vi "Ramsey_Tau_manipulation.vi"(8 "Dont Invert?":bool, 9 "Numeric 2":i32, 10 "Numeric":i32, 11 "Step Size":dbl format="%#_13g") -> (2 "x+y":dbl)   [LabVIEW 2024]
uses:
  <vilib>/Utility/error.llb/DialogTypeEnum.ctl
  SpinCore_API_file_location.vi
panel:
  out "x+y 4":dbl
  out "x+y 3":dbl
  out "output array 2":T1(array[cluster])
  out "output array":T1(array[cluster])
  in  "Instructions":T1(array[cluster])=[{"Instruct Data"=0, "Op Code"=0, "Flags"=[FALSE, FALSE, TRUE, FALSE, FALSE, FALSE, FALSE, TRUE, FALSE, FALSE, FALSE, FALSE, FALSE, FALSE, FALSE, FALSE, FALSE, FALSE, FALSE, FALSE, FALSE, FALSE, FALSE, TRUE], "Comments"="0 triggers", "Time (s)"=1e-07}, {"Instruct Data"=0, "Op Code"=0, "Flags"=[FALSE, FALSE, FALSE, FALSE, FALSE, FALSE, FALSE, TRUE, FALSE, FALSE, FALSE, FALSE, FALSE, FALSE, FALSE, FALSE, FALSE, FALSE, FALSE, FALSE, FALSE, FALSE, FALSE, FALSE], "Comments"="1Dark", "Time (s)"=6e-06}, {"Instruct Data"=0, "Op Code"=0, "Flags"=[TRUE, FALSE, FALSE, TRUE, FALSE, FALSE, FALSE, TRUE, FALSE, FALSE, FALSE, FALSE, FALSE, FALSE, FALSE, FALSE, FALSE, FALSE, FALSE, FALSE, FALSE, FALSE, FALSE, FALSE], "Comments"="2 pi/2", "Time (s)"=6.9e-08}, {"Instruct Data"=0, "Op Code"=0, "Flags"=[FALSE, FALSE, FALSE, FALSE, FALSE, FALSE, FALSE, TRUE, FALSE, FALSE, FALSE, FALSE, FALSE, FALSE, FALSE, FALSE, FALSE, FALSE, FALSE, FALSE, FALSE, FALSE, FALSE, FALSE], "Comments"="3 tau", "Time (s)"=1e-08}, {"Instruct Data"=0, "Op Code"=0, "Flags"=[TRUE, FALSE, FALSE, TRUE, FALSE, FALSE, FALSE, TRUE, FALSE, FALSE, FALSE, FALSE, FALSE, FALSE, FALSE, FALSE, FALSE, FALSE, FALSE, FALSE, FALSE, FALSE, FALSE, FALSE], "Comments"="4 pi/2", "Time (s)"=6.9e-08}, {"Instruct Data"=0, "Op Code"=0, "Flags"=[FALSE, TRUE, FALSE, FALSE, FALSE, FALSE, FALSE, TRUE, FALSE, FALSE, FALSE, FALSE, FALSE, FALSE, FALSE, FALSE, FALSE, FALSE, FALSE, FALSE, FALSE, FALSE, FALSE, FALSE], "Comments"="5 AOM Buffer", "Time (s)"=5e-07}, {"Instruct Data"=0, "Op Code"=0, "Flags"=[FALSE, TRUE, FALSE, FALSE, FALSE, FALSE, FALSE, FALSE, FALSE, FALSE, FALSE, FALSE, FALSE, FALSE, FALSE, FALSE, FALSE, FALSE, FALSE, FALSE, FALSE, FALSE, FALSE, FALSE], "Comments"="6 inhibit off", "Time (s)"=5e-07}, {"Instruct Data"=0, "Op Code"=0, "Flags"=[FALSE, TRUE, FALSE, FALSE, FALSE, FALSE, FALSE, TRUE, FALSE, FALSE, FALSE, FALSE, FALSE, FALSE, FALSE, FALSE, FALSE, FALSE, FALSE, FALSE, FALSE, FALSE, FALSE, FALSE], "Comments"="7  AOM", "Time (s)"=6e-06}, {"Instruct Data"=0, "Op Code"=0, "Flags"=[FALSE, FALSE, FALSE, FALSE, FALSE, FALSE, FALSE, TRUE, FALSE, FALSE, FALSE, FALSE, FALSE, FALSE, FALSE, FALSE, FALSE, FALSE, FALSE, FALSE, FALSE, FALSE, FALSE, FALSE], "Comments"="8 Dark", "Time (s)"=5e-06}, {"Instruct Data"=0, "Op Code"=0, "Flags"=[FALSE, TRUE, FALSE, FALSE, FALSE, FALSE, FALSE, TRUE, FALSE, FALSE, FALSE, FALSE, FALSE, FALSE, FALSE, FALSE, FALSE, FALSE, FALSE, FALSE, FALSE, FALSE, FALSE, FALSE], "Comments"="9AOM delay", "Time (s)"=5e-07}, {"Instruct Data"=0, "Op Code"=0, "Flags"=[FALSE, TRUE, FALSE, FALSE, FALSE, FALSE, FALSE, FALSE, FALSE, FALSE, FALSE, FALSE, FALSE, FALSE, FALSE, FALSE, FALSE, FALSE, FALSE, FALSE, FALSE, FALSE, FALSE, FALSE], "Comments"="10 inhibit off", "Time (s)"=5e-07}, {"Instruct Data"=0, "Op Code"=6, "Flags"=[FALSE, TRUE, FALSE, FALSE, FALSE, FALSE, FALSE, TRUE, FALSE, FALSE, FALSE, FALSE, FALSE, FALSE, FALSE, FALSE, FALSE, FALSE, FALSE, FALSE, FALSE, FALSE, FALSE, FALSE], "Comments"="11 AOM", "Time (s)"=6e-06}, {"Instruct Data"=0, "Op Code"=6, "Flags"=[FALSE, FALSE, FALSE, FALSE, FALSE, FALSE, FALSE, FALSE, FALSE, FALSE, FALSE, FALSE, FALSE, FALSE, FALSE, FALSE, FALSE, FALSE, FALSE, FALSE, FALSE, FALSE, FALSE, FALSE], "Comments"="12", "Time (s)"=1e-06}] {"Time (s)" format="%.3p"; "Op Code" items=["Continue", "Stop", "Loop", "End Loop", "JSR", "RTS", "Branch", "Long Delay", "Wait"]}
  in  "# of Instructions":u32=12
  in  "clock_freq (MHz)":dbl=500.0
  # "1)MW\n2)AOM\n3)SR400 Trig\n4) I\n5)Q\n8) Inhibit\n24) Oscillocope trig"
  # "1"
  # "2"
  # "3"
  # "4"
  # "5"
  # "6"
  # "7"
  # "8"
  # "9"
  # "10"
  # "11"
  # "12"
  # "13"
  # "14"
  # "15"
  # "16"
  # "17"
  # "18"
  # "19"
  # "20"
  # "21"
  # "22"
  # "23"
  # "24"
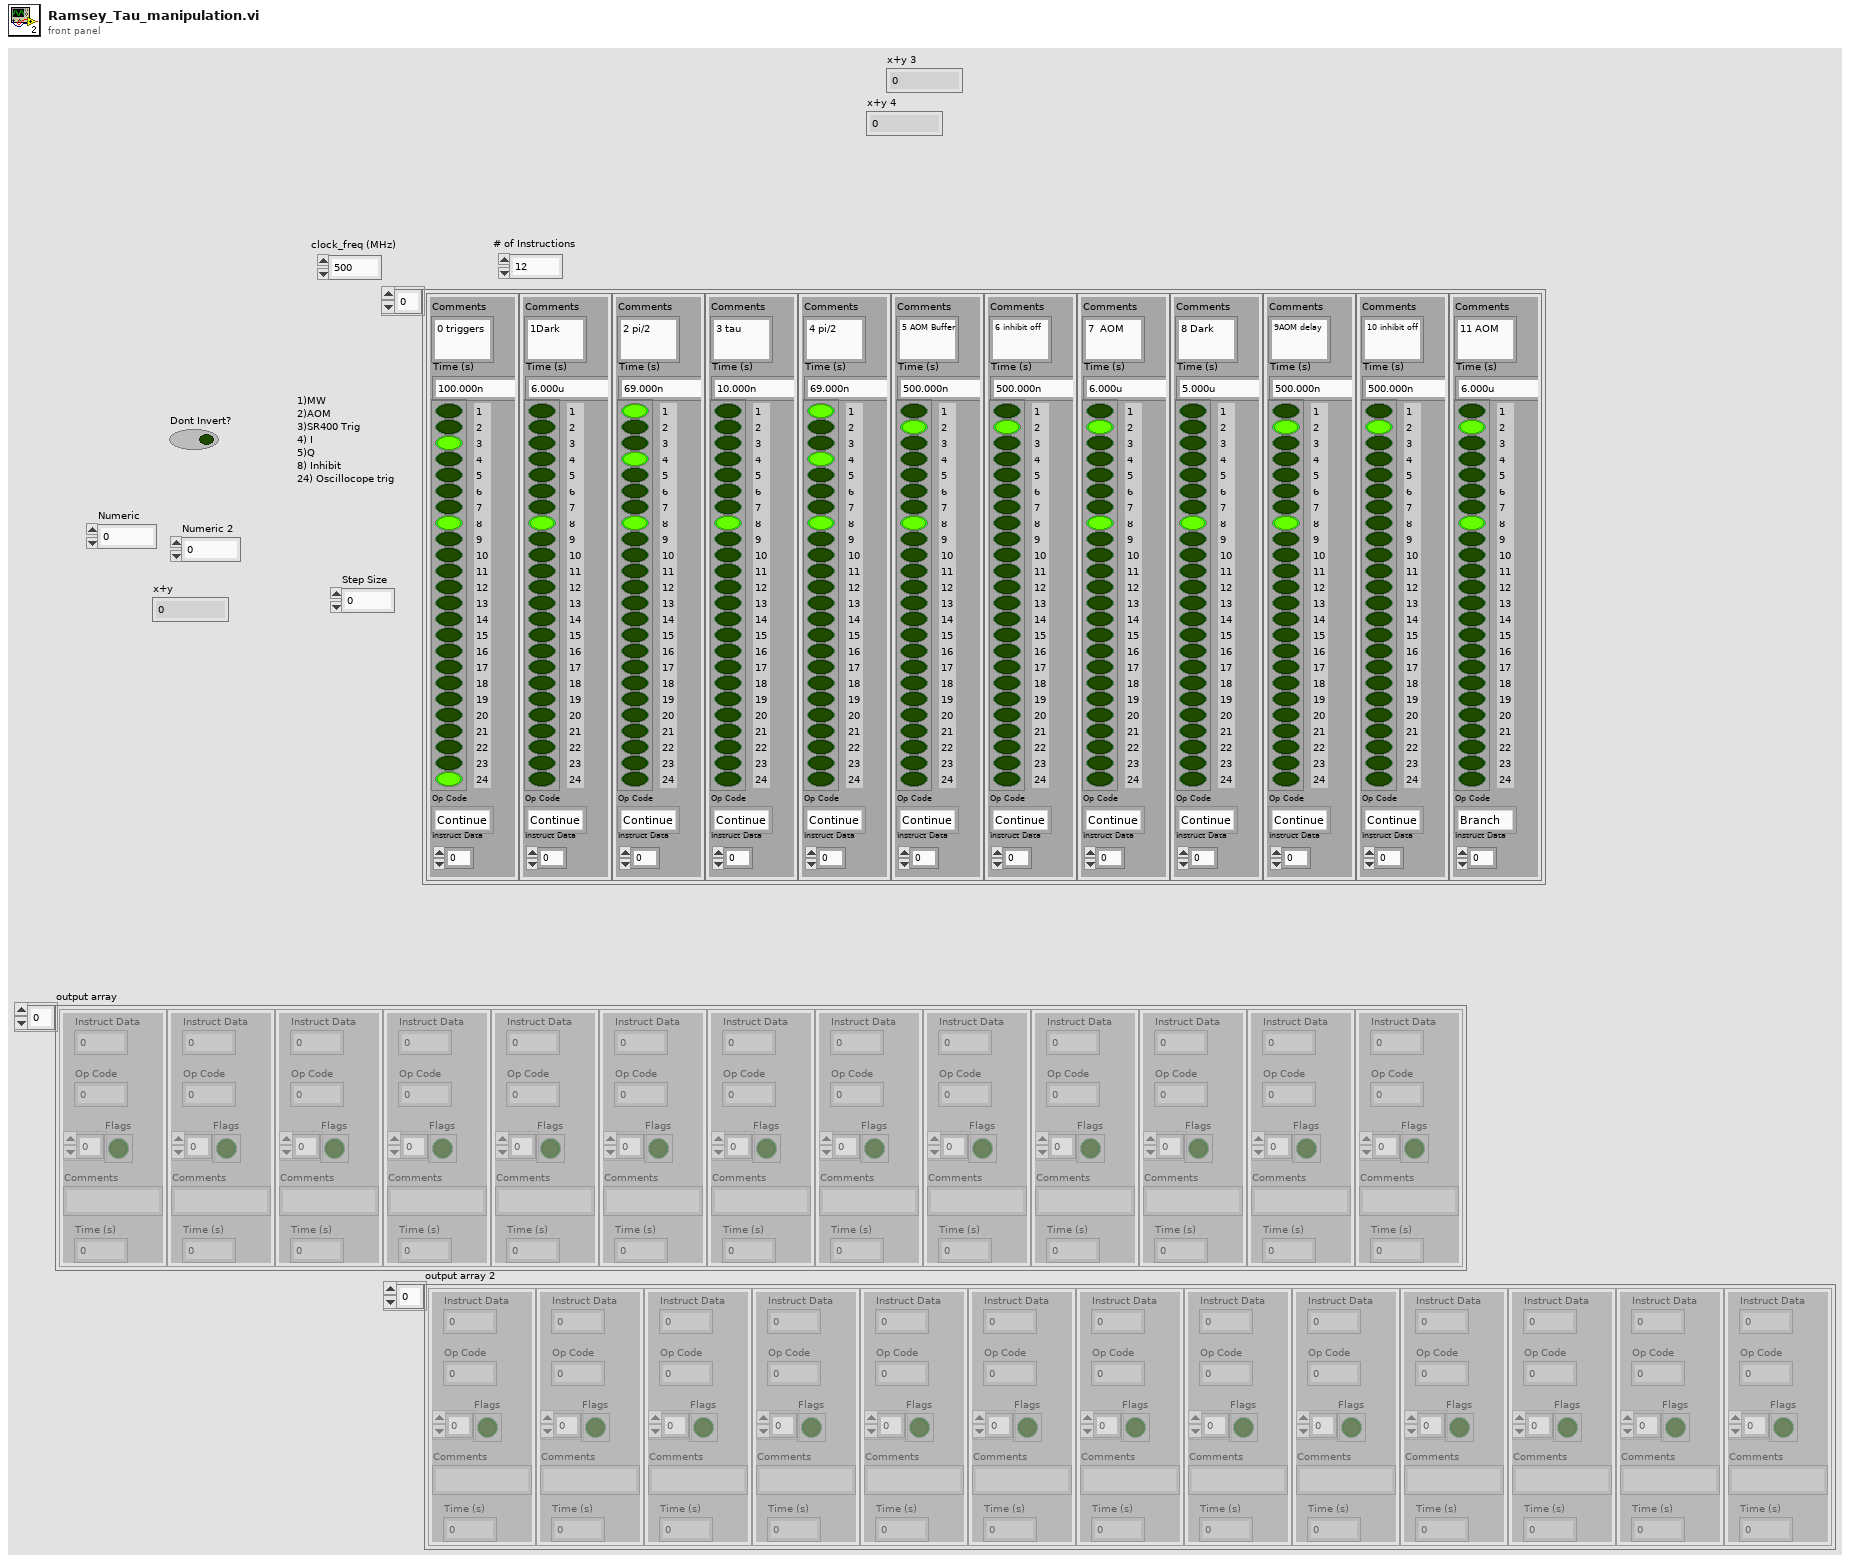
[diagram p1: front panel]
types:
  T1 = cluster{"Instruct Data":i32, "Op Code":i32, "Flags":bool[], "Comments":string, "Time (s)":dbl}[]
  T2 = typedef "DialogTypeEnum.ctl" = enum16{"no dialog", "OK message", "continue or stop message", "auto error handling dialog", "OK message + warnings", "continue/stop + warnings"}
  T3 = enum16{"Pulse Program", "Frequency Registers", "TX Phase Registers", "RX Phase Registers"}
  T4 = cluster{"Instruct Data":i32, "Op Code":i32, "Flags":bool[], "Comments":string, "Time (s)":dbl}
  T5 = cluster{"Instruct Data":i32, "Op Code":i32, "Flags":bool[], "Comments":string, dbl}
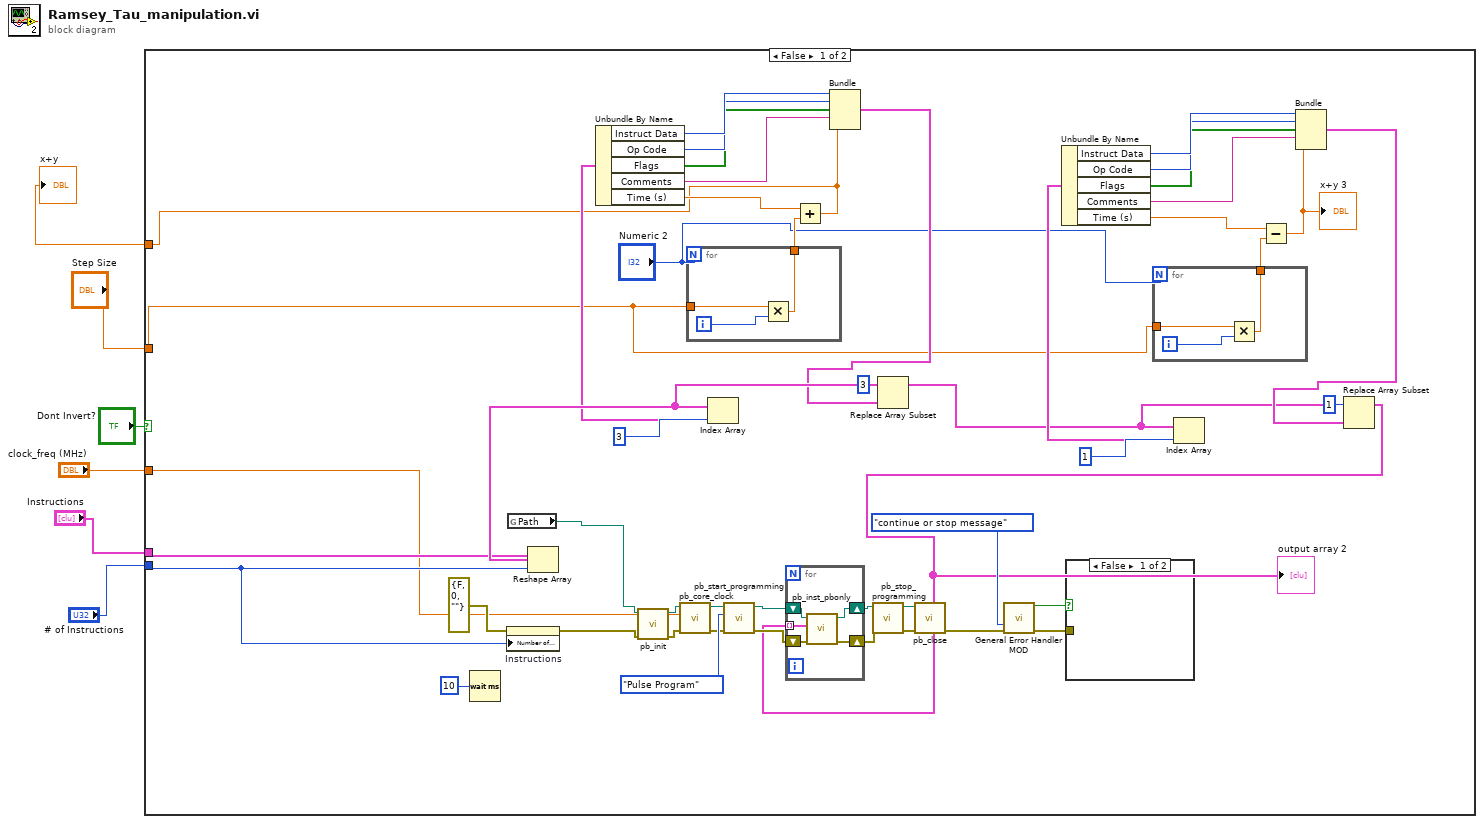
[diagram p0: block diagram]
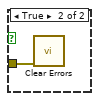
[diagram p2: hidden frame]
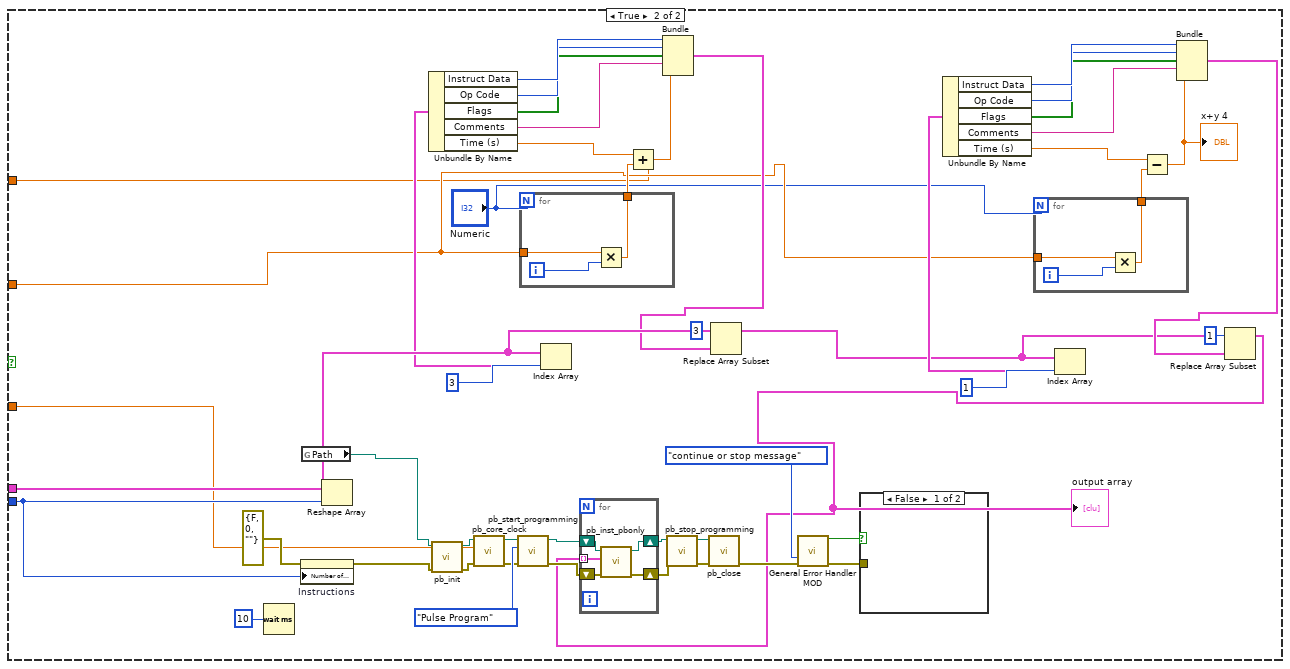
[diagram p3: hidden frame]
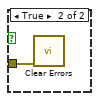
[diagram p4: hidden frame]
diagram:
  n1 = case shown="False" "Dont Invert?" {
    tunnel: "Instructions" -> [w25 w86]
    tunnel: "# of Instructions" -> [w24 w85]
    tunnel: "clock_freq (MHz)" -> [w23 w84]
    tunnel: "Step Size" -> [w9 w72]
    tunnel: [w7 w68] -> w1
    frame False {
      n2 = Wait (ms)(milliseconds to wait=u32 10) -> ()  [unwired: 1 out]
      n3 = property on="Instructions" class="Arr (strict)"(error in=errorcluster {"status"=FALSE, "code"=0, "source"=""} ("error in (no error)"), "Number of Columns"=w24) -> (error out=w30:errorcluster)  [unwired: 1 in, 1 out]
      n4 = global read "SpinCore_API_file_location.vi" "Path"() -> (w31:path)
      n5 = Reshape Array "Reshape Array"(w25, w24) -> (w36:T1)
      n6 = call "pb_init.vi"("error in (no error)"=w30, "path in"=w31) -> ("error out"=w29:errorcluster, "path out"=w28:path)  [unwired: 8 in]
      n7 = call "pb_core_clock.vi"("error in (no error)"=w29, "clock_freq (MHz)"=w23, "path in"=w28) -> ("error out"=w44:errorcluster, "path out"=w45:path)  [unwired: 7 in]
      n8 = for {
        N: "Numeric 2" -> [_]
        tunnel: [w60] -> w32
        tunnel: w9 -> [w59]
        i -> [w61]
        n9 = Multiply(x=w59, y=w61) -> (x*y=w60:dbl)
      }
      n10 = Index Array "Index Array"(array=w36, index=3) -> (element=w35:T4)
      n11 = Unbundle By Name "Unbundle By Name"(w35) -> ("Instruct Data"=w41:i32, "Op Code"=w40:i32, "Flags"=w39:bool[], "Comments"=w38:string, "Time (s)"=w37:dbl)
      n12 = call "pb_start_programming.vi"("error in (no error)"=w44, "Device"=T3."Pulse Program", "path in"=w45) -> ("error out"=w51:errorcluster, "path out"=w55:path)  [unwired: 1 in, 6 out]
      n13 = Add(x=w37, y=w32) -> (x+y=w7:dbl)
      n14 = Bundle("Instruct Data"=w41, "Op Code"=w40, "Flags"=w39, "Comments"=w38, w7) -> (w33:T5)  [unwired: 1 in]
      n15 = Replace Array Subset "Replace Array Subset"(array=w36, new element=w33, index=3) -> (w11:T1)
      n16 = for {
        N: "Numeric 2" -> [_]
        tunnel: [w57] -> w12
        tunnel: w9 -> [w56]
        i -> [w58]
        n17 = Multiply(x=w56, y=w58) -> (x*y=w57:dbl)
      }
      n18 = Index Array "Index Array"(array=w11, index=1) -> (element=w15:T4)
      n19 = Unbundle By Name "Unbundle By Name"(w15) -> ("Instruct Data"=w21:i32, "Op Code"=w20:i32, "Flags"=w19:bool[], "Comments"=w18:string, "Time (s)"=w17:dbl)
      n20 = Subtract(x=w17, y=w12) -> (x-y=w16:dbl)
      "x+y 3" <- w16
      n21 = Bundle("Instruct Data"=w21, "Op Code"=w20, "Flags"=w19, "Comments"=w18, w16) -> (w13:T5)  [unwired: 1 in]
      n22 = Replace Array Subset "Replace Array Subset"(array=w11, new element=w13, index=1) -> (w10:T1)
      "output array 2" <- w10
      n23 = for {
        tunnel: w10 -> [w64] mode=indexing
        shift-right: [w66] -> w53
        shift-left: w55 -> [w67]
        shift-right: [w63] -> w50
        shift-left: w51 -> [w65]
        n24 = call "pb_inst_pbonly.vi"("error in (no error)"=w65, "PB Instruction"=w64, "path in"=w67) -> ("error out"=w63:errorcluster, "path out"=w66:path)  [unwired: 2 in, 5 out]
      }
      n25 = call "pb_stop_programming.vi"("error in (no error)"=w50, "path in"=w53) -> ("error out"=w49:errorcluster, "path out"=w54:path)  [unwired: 1 in, 7 out]
      n26 = call "pb_close.vi"("error in (no error)"=w49, "path in"=w54) -> ("error out"=w43:errorcluster)  [unwired: 9 out]
      n27 = call "General Error Handler MOD.vi"("type of dialog (OK msg:1)"=DialogTypeEnum."continue or stop message", "error in (no error)"=w43) -> ("STOP?"=w46:bool, "error out"=w47:errorcluster)  [unwired: 12 out]
      n28 = case shown="False" w46 {
        tunnel: w47 -> [_ w62]
        frame False {
        }
        frame True {
          n29 = call <vilib>:"Clear Errors.vi"("error in (no error)"=w62) -> ()  [unwired: 1 in, 6 out]
        }
      }
    }
    frame True {
      n30 = Wait (ms)(milliseconds to wait=u32 10) -> ()  [unwired: 1 out]
      n31 = property on="Instructions" class="Arr (strict)"(error in=errorcluster {"status"=FALSE, "code"=0, "source"=""} ("error in (no error)"), "Number of Columns"=w85) -> (error out=w91:errorcluster)  [unwired: 1 in, 1 out]
      n32 = global read "SpinCore_API_file_location.vi" "Path"() -> (w92:path)
      n33 = Reshape Array "Reshape Array"(w86, w85) -> (w97:T1)
      n34 = call "pb_init.vi"("error in (no error)"=w91, "path in"=w92) -> ("error out"=w90:errorcluster, "path out"=w89:path)  [unwired: 8 in]
      n35 = call "pb_core_clock.vi"("error in (no error)"=w90, "clock_freq (MHz)"=w84, "path in"=w89) -> ("error out"=w105:errorcluster, "path out"=w106:path)  [unwired: 7 in]
      n36 = call "pb_start_programming.vi"("error in (no error)"=w105, "Device"=T3."Pulse Program", "path in"=w106) -> ("error out"=w112:errorcluster, "path out"=w116:path)  [unwired: 1 in, 6 out]
      n37 = for {
        N: "Numeric" -> [_]
        tunnel: [w121] -> w93
        tunnel: w72 -> [w120]
        i -> [w122]
        n38 = Multiply(x=w120, y=w122) -> (x*y=w121:dbl)
      }
      n39 = Index Array "Index Array"(array=w97, index=3) -> (element=w96:T4)
      n40 = Unbundle By Name "Unbundle By Name"(w96) -> ("Instruct Data"=w102:i32, "Op Code"=w101:i32, "Flags"=w100:bool[], "Comments"=w99:string, "Time (s)"=w98:dbl)
      n41 = Add(x=w98, y=w93) -> (x+y=w68:dbl)
      n42 = Bundle("Instruct Data"=w102, "Op Code"=w101, "Flags"=w100, "Comments"=w99, w68) -> (w94:T5)  [unwired: 1 in]
      n43 = Replace Array Subset "Replace Array Subset"(array=w97, new element=w94, index=3) -> (w70:T1)
      n44 = for {
        N: "Numeric" -> [_]
        tunnel: [w118] -> w73
        tunnel: w72 -> [w117]
        i -> [w119]
        n45 = Multiply(x=w117, y=w119) -> (x*y=w118:dbl)
      }
      n46 = Index Array "Index Array"(array=w70, index=1) -> (element=w76:T4)
      n47 = Unbundle By Name "Unbundle By Name"(w76) -> ("Instruct Data"=w82:i32, "Op Code"=w81:i32, "Flags"=w80:bool[], "Comments"=w79:string, "Time (s)"=w78:dbl)
      n48 = Subtract(x=w78, y=w73) -> (x-y=w77:dbl)
      "x+y 4" <- w77
      n49 = Bundle("Instruct Data"=w82, "Op Code"=w81, "Flags"=w80, "Comments"=w79, w77) -> (w74:T5)  [unwired: 1 in]
      n50 = Replace Array Subset "Replace Array Subset"(array=w70, new element=w74, index=1) -> (w69:T1)
      "output array" <- w69
      n51 = for {
        tunnel: w69 -> [w125] mode=indexing
        shift-right: [w127] -> w114
        shift-left: w116 -> [w128]
        shift-right: [w124] -> w111
        shift-left: w112 -> [w126]
        n52 = call "pb_inst_pbonly.vi"("error in (no error)"=w126, "PB Instruction"=w125, "path in"=w128) -> ("error out"=w124:errorcluster, "path out"=w127:path)  [unwired: 2 in, 5 out]
      }
      n53 = call "pb_stop_programming.vi"("error in (no error)"=w111, "path in"=w114) -> ("error out"=w110:errorcluster, "path out"=w115:path)  [unwired: 1 in, 7 out]
      n54 = call "pb_close.vi"("error in (no error)"=w110, "path in"=w115) -> ("error out"=w104:errorcluster)  [unwired: 9 out]
      n55 = call "General Error Handler MOD.vi"("type of dialog (OK msg:1)"=DialogTypeEnum."continue or stop message", "error in (no error)"=w104) -> ("STOP?"=w107:bool, "error out"=w108:errorcluster)  [unwired: 12 out]
      n56 = case shown="False" w107 {
        tunnel: w108 -> [_ w123]
        frame False {
        }
        frame True {
          n57 = call <vilib>:"Clear Errors.vi"("error in (no error)"=w123) -> ()  [unwired: 1 in, 6 out]
        }
      }
    }
  }
  "x+y" <- w1
